vi "Test.vi"   [LabVIEW 2019]
doc: "This VI is called when test mode begins, and will automatically be terminated when it ends. You can add manual or automatic tests and invoke them from the dashboard."
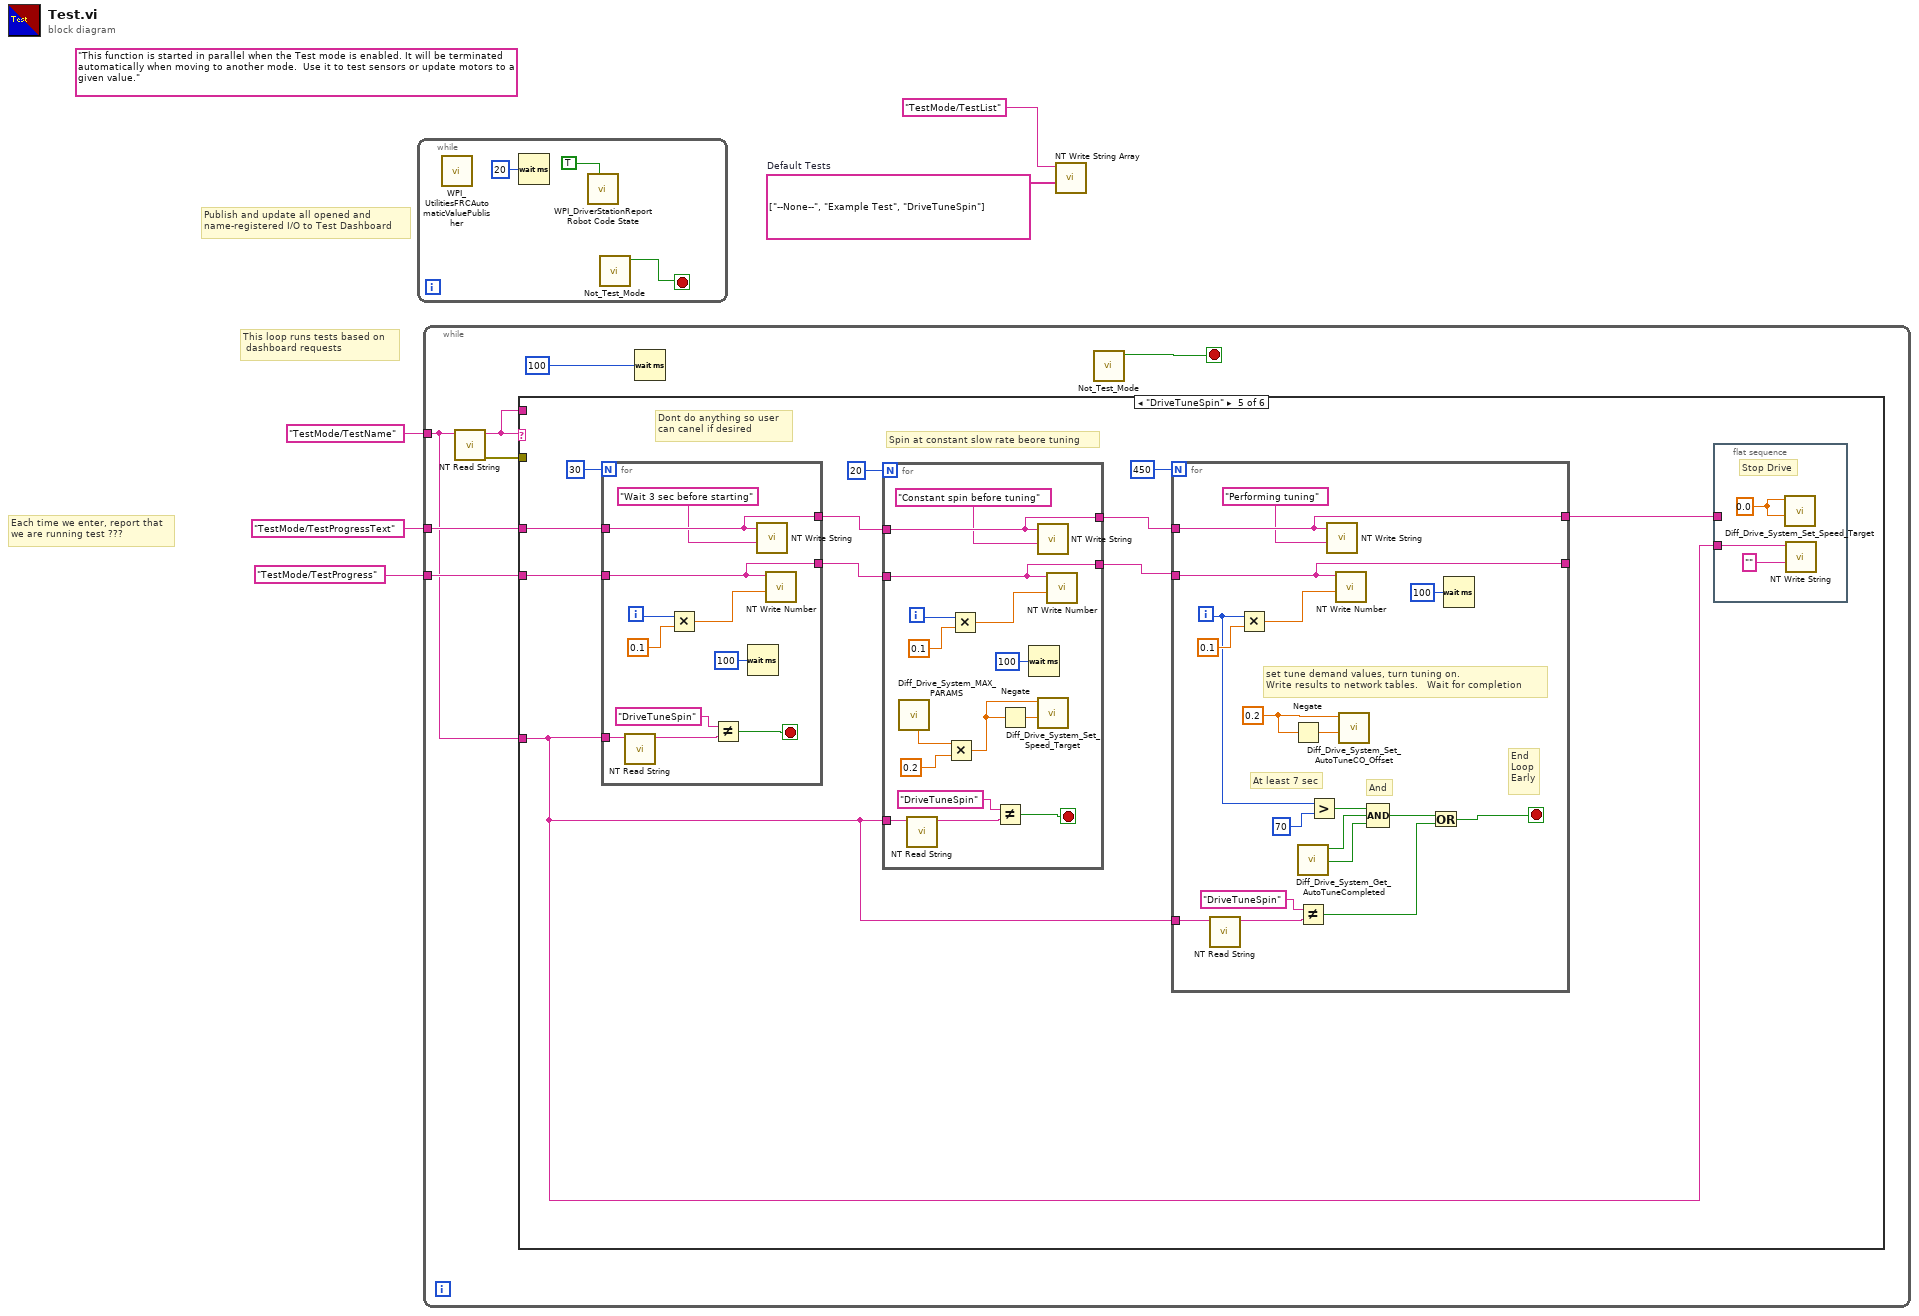
[diagram p0: block diagram]
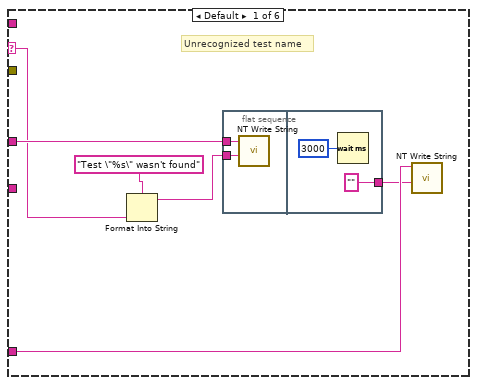
[diagram p2: hidden frame]
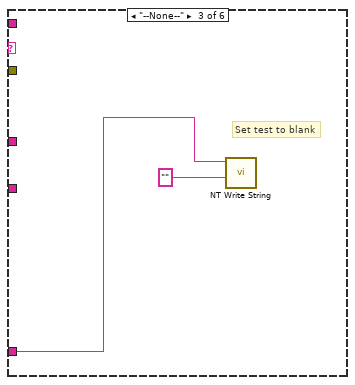
[diagram p4: hidden frame]
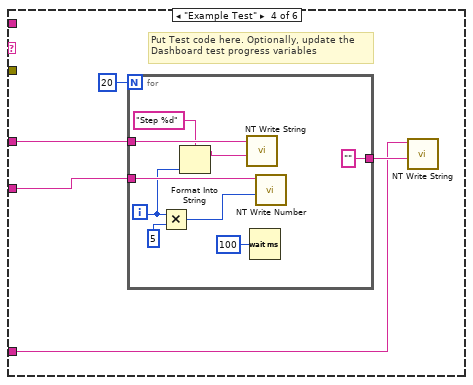
[diagram p5: hidden frame]
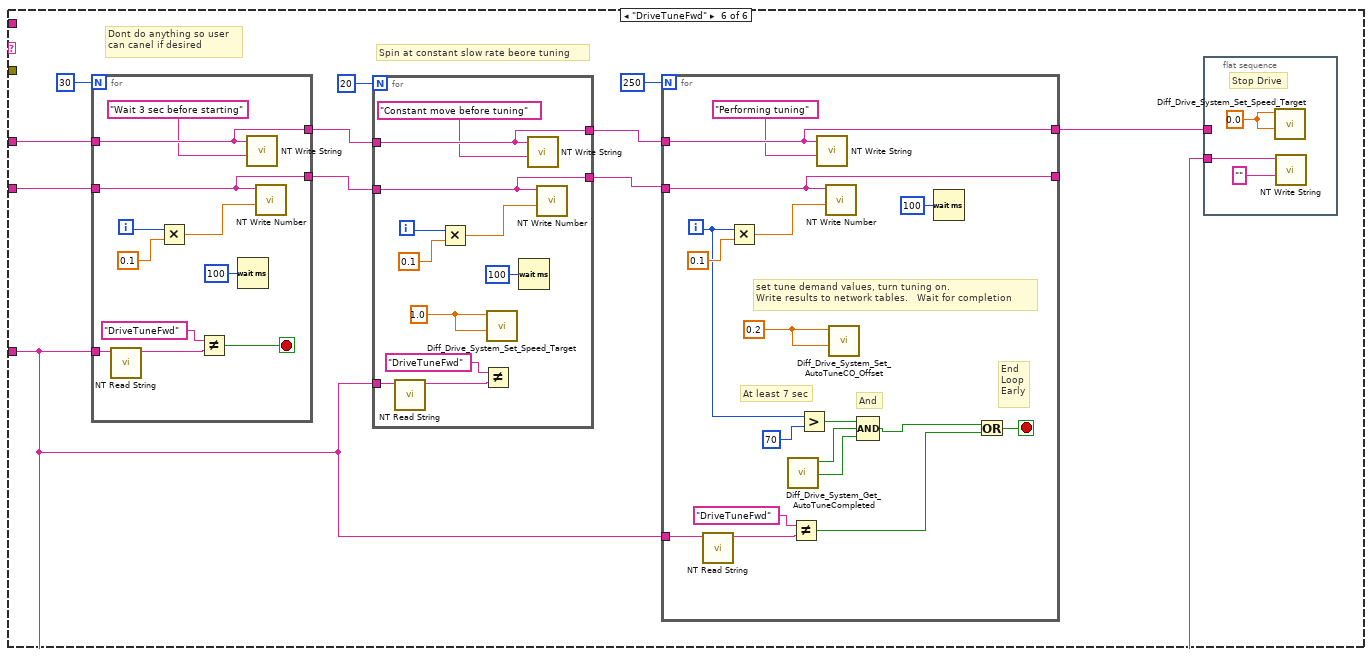
[diagram p6: hidden frame]
diagram:
  w2 = string[] ["--None--", "Example Test", "DriveTuneSpin"]  # Default Tests
  (unwired) "This function is started in parallel when the Test mode is enabled. It will be terminated automatically when moving to another mode.  Use it to test sensors or update motors to a given value."
  # "This loop runs tests based on \n dashboard requests"
  # "Publish and update all opened and\nname-registered I/O to Test Dashboard"
  # "Each time we enter, report that\nwe are running test ???"
  n1 = while {
    stop <- w6 stop-if-true
    n2 = call <vilib>:"WPI_UtilitiesFRCAutomaticValuePublisher.vi"() -> ()  [unwired: 12 in]
    n3 = Wait (ms)(milliseconds to wait=u32 20) -> ()  [unwired: 1 out]
    n4 = call <vilib>:"WPI_DriverStationReport Robot Code State.vi"("Test"=TRUE ("Autonomous")) -> ()  [unwired: 10 in, 1 out]
    n5 = call "Not_Test_Mode.vi"() -> ("NOT TEST MODE"=w6:bool)  [unwired: 11 in]
  }
  n6 = while {
    tunnel: "TestMode/TestName" ("Name") -> [w11]
    tunnel: "TestMode/TestProgressText" ("Name") -> [w14]
    tunnel: "TestMode/TestProgress" ("Name") -> [w13]
    stop <- w9 stop-if-true
    n7 = call <vilib>:"NT Read String.vi"("Name"=w11) -> ("error out"=w10:errorcluster, "String"=w12:string)  [unwired: 9 in]
    n8 = case shown="\"DriveTuneSpin\"" w12 {
      selector: w12 -> [w20 _ _ _ _ _]
      tunnel: w11 -> [w17 _ w27 w28 w42 w101]
      tunnel: w14 -> [w21 _ _ w31 w51 w110]
      tunnel: w13 -> [_ _ _ w32 w52 w111]
      tunnel: w12 -> [_ _ _ _ _ _]
      tunnel: w10 -> [_ _ _ _ _ _]
      frame Default {
        # "Unrecognized test name"
        n9 = Format Into String(format string="Test \"%s\" wasn't found" ("Name"), w20) -> (resulting string=w19:string)  [unwired: 2 in, 1 out]
        n10 = flat-sequence {
          tunnel: w21 -> [w22]
          tunnel: w19 -> [w23]
          tunnel: ["" ("Name")] -> w16
          frame #0 {
            n11 = call <vilib>:"NT Write String.vi"("String"=w23, "Name"=w22) -> ()  [unwired: 9 in, 1 out]
          }
          frame #1 {
            n12 = Wait (ms)(milliseconds to wait=u32 3000) -> ()  [unwired: 1 out]
          }
        }
        n13 = call <vilib>:"NT Write String.vi"("String"=w16, "Name"=w17) -> ()  [unwired: 9 in, 1 out]
      }
      frame "" {
        # "No test to run"
      }
      frame "--None--" {
        # "Set test to blank"
        n14 = call <vilib>:"NT Write String.vi"("String"="" ("Name"), "Name"=w27) -> ()  [unwired: 9 in, 1 out]
      }
      frame "Example Test" {
        # "Put Test code here. Optionally, update the\nDashboard test progress variables"
        n15 = for {
          N: 20 -> [_]
          tunnel: w32 -> [w41]
          tunnel: w31 -> [w39]
          tunnel: ["" ("String")] -> w29
          i -> [w36]
          n16 = Multiply(x=w36, y=u32 5 ("milliseconds to wait")) -> (x*y=w37:u32)
          n17 = Format Into String(format string="Step %d", w36) -> (resulting string=w34:string)  [unwired: 2 in, 1 out]
          n18 = call <vilib>:"NT Write String.vi"("String"=w34, "Name"=w39) -> ()  [unwired: 9 in, 1 out]
          n19 = Wait (ms)(milliseconds to wait=u32 100) -> ()  [unwired: 1 out]
          n20 = call <vilib>:"NT Write Number.vi"("Numeric"=w37, "Name"=w41) -> ()  [unwired: 9 in, 1 out]
        }
        n21 = call <vilib>:"NT Write String.vi"("String"=w29, "Name"=w28) -> ()  [unwired: 9 in, 1 out]
      }
      frame "DriveTuneSpin" {
        # "Spin at constant slow rate beore tuning"
        # "Dont do anything so user\ncan canel if desired"
        n22 = for {
          N: 30 -> [_]
          tunnel: w52 -> [w95]
          tunnel: w51 -> [w96]
          tunnel: [w96] -> w48
          tunnel: [w95] -> w47
          tunnel: w42 -> [w93]
          i -> [w97]
          stop <- w90 stop-if-true
          n23 = call <vilib>:"NT Read String.vi"("Name"=w93) -> ("String"=w91:string)  [unwired: 9 in, 1 out]
          n24 = Multiply(x=w97, y=0.1) -> (x*y=w98:dbl)
          n25 = Not Equal?(x="DriveTuneSpin" ("format string"), y=w91) -> (x != y?=w90:bool)
          n26 = Wait (ms)(milliseconds to wait=u32 100) -> ()  [unwired: 1 out]
          n27 = call <vilib>:"NT Write String.vi"("String"="Wait 3 sec before starting" ("format string"), "Name"=w96) -> ()  [unwired: 9 in, 1 out]
          n28 = call <vilib>:"NT Write Number.vi"("Numeric"=w98, "Name"=w95) -> ()  [unwired: 9 in, 1 out]
        }
        n29 = for {
          N: 20 -> [_]
          tunnel: w47 -> [w84]
          tunnel: w48 -> [w85]
          tunnel: [w85] -> w45
          tunnel: [w84] -> w44
          tunnel: w42 -> [w75]
          i -> [w86]
          stop <- w76 stop-if-true
          n30 = call "Diff_Drive_System_MAX_PARAMS.vi"() -> ("Max Drive Speed Ft/Sec"=w83:dbl)  [unwired: 9 in, 2 out]
          n31 = call <vilib>:"NT Read String.vi"("Name"=w75) -> ("String"=w77:string)  [unwired: 9 in, 1 out]
          n32 = Multiply(x=w83, y=0.2) -> (x*y=w80:dbl)
          n33 = Multiply(x=w86, y=0.1) -> (x*y=w87:dbl)
          n34 = Not Equal?(x="DriveTuneSpin" ("format string"), y=w77) -> (x != y?=w76:bool)
          n35 = Negate(x=w80) -> (-x=w81:dbl)
          n36 = Wait (ms)(milliseconds to wait=u32 100) -> ()  [unwired: 1 out]
          n37 = call <vilib>:"NT Write String.vi"("String"="Constant spin before tuning" ("format string"), "Name"=w85) -> ()  [unwired: 9 in, 1 out]
          n38 = call "Diff_Drive_System_Set_Speed_Target.vi"("Right Speed Target FT/S"=w81, "Left Speed Target FT/S"=w80) -> ()  [unwired: 10 in]
          n39 = call <vilib>:"NT Write Number.vi"("Numeric"=w87, "Name"=w84) -> ()  [unwired: 9 in, 1 out]
        }
        n40 = for {
          N: 450 -> [_]
          tunnel: w44 -> [w70]
          tunnel: w45 -> [w71]
          tunnel: [w71] -> w43
          tunnel: [w70] -> _
          tunnel: w42 -> [w59]
          i -> [w66]
          stop <- w56 stop-if-true
          w68 = 0.2 ("Left CO Offset")
          # "End\nLoop\nEarly"
          # "And"
          # "At least 7 sec"
          # "set tune demand values, turn tuning on.\nWrite results to network tables.   Wait for completion"
          n41 = call <vilib>:"NT Read String.vi"("Name"=w59) -> ("String"=w60:string)  [unwired: 9 in, 1 out]
          n42 = Multiply(x=w66, y=0.1) -> (x*y=w72:dbl)
          n43 = Negate(x=w68) -> (-x=w67:dbl)
          n44 = call "Diff_Drive_System_Get_AutoTuneCompleted.vi"() -> ("AutoTune Complete Right"=w62:bool, "AutoTune Complete Left"=w63:bool)  [unwired: 10 in]
          n45 = Not Equal?(x="DriveTuneSpin" ("format string"), y=w60) -> (x != y?=w57:bool)
          n46 = Greater?(x=w66, y=70) -> (0:w64:bool)
          n47 = call <vilib>:"NT Write String.vi"("String"="Performing tuning" ("format string"), "Name"=w71) -> ()  [unwired: 9 in, 1 out]
          n48 = call <vilib>:"NT Write Number.vi"("Numeric"=w72, "Name"=w70) -> ()  [unwired: 9 in, 1 out]
          n49 = call "Diff_Drive_System_Set_AutoTuneCO_Offset.vi"("Right CO Offset"=w67, "Left CO Offset"=w68) -> ()  [unwired: 10 in]
          n50 = Compound Arithmetic op=AND(w64, w63, w62) -> (w58:bool)
          n51 = Or(x=w58, y=w57) -> (x .or. y?=w56:bool)
          n52 = Wait (ms)(milliseconds to wait=u32 100) -> ()  [unwired: 1 out]
        }
        n53 = flat-sequence {
          tunnel: w43 -> [_]
          tunnel: w42 -> [w54]
          frame #0 {
            w53 = 0.0 ("Left Speed Target FT/S")
            # "Stop Drive"
            n54 = call "Diff_Drive_System_Set_Speed_Target.vi"("Right Speed Target FT/S"=w53, "Left Speed Target FT/S"=w53) -> ()  [unwired: 10 in]
            n55 = call <vilib>:"NT Write String.vi"("String"="", "Name"=w54) -> ()  [unwired: 9 in, 1 out]
          }
        }
      }
      frame "DriveTuneFwd" {
        # "Spin at constant slow rate beore tuning"
        # "Dont do anything so user\ncan canel if desired"
        n56 = for {
          N: 30 -> [_]
          tunnel: w111 -> [w149]
          tunnel: w110 -> [w150]
          tunnel: [w150] -> w107
          tunnel: [w149] -> w106
          tunnel: w101 -> [w145]
          i -> [w151]
          stop <- w144 stop-if-true
          n57 = call <vilib>:"NT Read String.vi"("Name"=w145) -> ("String"=w146:string)  [unwired: 9 in, 1 out]
          n58 = Multiply(x=w151, y=0.1) -> (x*y=w152:dbl)
          n59 = Not Equal?(x="DriveTuneFwd" ("format string"), y=w146) -> (x != y?=w144:bool)
          n60 = Wait (ms)(milliseconds to wait=u32 100) -> ()  [unwired: 1 out]
          n61 = call <vilib>:"NT Write String.vi"("String"="Wait 3 sec before starting" ("format string"), "Name"=w150) -> ()  [unwired: 9 in, 1 out]
          n62 = call <vilib>:"NT Write Number.vi"("Numeric"=w152, "Name"=w149) -> ()  [unwired: 9 in, 1 out]
        }
        n63 = for {
          N: 20 -> [_]
          tunnel: w106 -> [w138]
          tunnel: w107 -> [w139]
          tunnel: [w139] -> w104
          tunnel: [w138] -> w103
          tunnel: w101 -> [w133]
          i -> [w140]
          w136 = 1.0 ("y")
          n64 = call <vilib>:"NT Read String.vi"("Name"=w133) -> ("String"=w134:string)  [unwired: 9 in, 1 out]
          n65 = Multiply(x=w140, y=0.1) -> (x*y=w141:dbl)
          n66 = Not Equal?(x="DriveTuneFwd" ("format string"), y=w134) -> ()  [unwired: 1 out]
          n67 = call "Diff_Drive_System_Set_Speed_Target.vi"("Right Speed Target FT/S"=w136, "Left Speed Target FT/S"=w136) -> ()  [unwired: 10 in]
          n68 = Wait (ms)(milliseconds to wait=u32 100) -> ()  [unwired: 1 out]
          n69 = call <vilib>:"NT Write String.vi"("String"="Constant move before tuning" ("format string"), "Name"=w139) -> ()  [unwired: 9 in, 1 out]
          n70 = call <vilib>:"NT Write Number.vi"("Numeric"=w141, "Name"=w138) -> ()  [unwired: 9 in, 1 out]
        }
        n71 = for {
          N: 250 -> [_]
          tunnel: w103 -> [w128]
          tunnel: w104 -> [w129]
          tunnel: [w129] -> w102
          tunnel: [w128] -> _
          tunnel: w101 -> [w118]
          i -> [w126]
          stop <- w117 stop-if-true
          w121 = 0.2 ("Left CO Offset")
          # "End\nLoop\nEarly"
          # "And"
          # "At least 7 sec"
          # "set tune demand values, turn tuning on.\nWrite results to network tables.   Wait for completion"
          n72 = call <vilib>:"NT Read String.vi"("Name"=w118) -> ("String"=w119:string)  [unwired: 9 in, 1 out]
          n73 = Multiply(x=w126, y=0.1) -> (x*y=w130:dbl)
          n74 = call "Diff_Drive_System_Get_AutoTuneCompleted.vi"() -> ("AutoTune Complete Right"=w122:bool, "AutoTune Complete Left"=w123:bool)  [unwired: 10 in]
          n75 = Not Equal?(x="DriveTuneFwd" ("format string"), y=w119) -> (x != y?=w115:bool)
          n76 = Greater?(x=w126, y=70) -> (0:w124:bool)
          n77 = call <vilib>:"NT Write String.vi"("String"="Performing tuning" ("format string"), "Name"=w129) -> ()  [unwired: 9 in, 1 out]
          n78 = call <vilib>:"NT Write Number.vi"("Numeric"=w130, "Name"=w128) -> ()  [unwired: 9 in, 1 out]
          n79 = call "Diff_Drive_System_Set_AutoTuneCO_Offset.vi"("Right CO Offset"=w121, "Left CO Offset"=w121) -> ()  [unwired: 10 in]
          n80 = Compound Arithmetic op=AND(w124, w123, w122) -> (w116:bool)
          n81 = Wait (ms)(milliseconds to wait=u32 100) -> ()  [unwired: 1 out]
          n82 = Or(x=w116, y=w115) -> (x .or. y?=w117:bool)
        }
        n83 = flat-sequence {
          tunnel: w102 -> [_]
          tunnel: w101 -> [w113]
          frame #0 {
            w112 = 0.0 ("Left Speed Target FT/S")
            # "Stop Drive"
            n84 = call "Diff_Drive_System_Set_Speed_Target.vi"("Right Speed Target FT/S"=w112, "Left Speed Target FT/S"=w112) -> ()  [unwired: 10 in]
            n85 = call <vilib>:"NT Write String.vi"("String"="", "Name"=w113) -> ()  [unwired: 9 in, 1 out]
          }
        }
      }
    }
    n86 = Wait (ms)(milliseconds to wait=u32 100) -> ()  [unwired: 1 out]
    n87 = call "Not_Test_Mode.vi"() -> ("NOT TEST MODE"=w9:bool)  [unwired: 11 in]
  }
  n88 = call <vilib>:"NT Write String Array.vi"("String Array"=w2, "Name"="TestMode/TestList") -> ()  [unwired: 9 in, 1 out]
